vi "RemoteVI Next Free Port.vi"(0 "used":u16[](array[numeric]), 1 "start":u16=8100) -> (4 "port":u16)   [LabVIEW 2020, in "RemoteVI.lvlib"]
doc: "The first port from start up that none of used has (RemoteVI Server suggests it for the next share, used being the ports of RemoteVI Status.vi). Pure. Reference: nextFreePort() in tools\\lib\\server-app.mjs."
uses:
  RemoteVI.lvlib
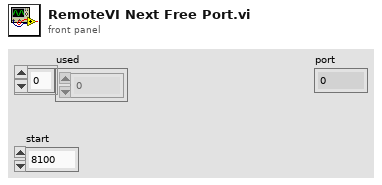
[diagram p1: front panel]
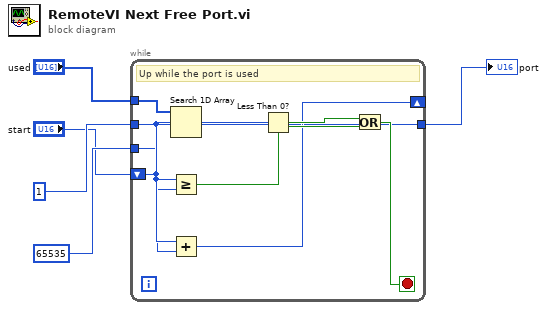
[diagram p0: block diagram]
diagram:
  n1 = while {
    tunnel: "used" -> [w6]
    tunnel: u16 1 -> [w7]
    tunnel: u16 65535 -> [w8]
    shift-right: [w10] -> _
    shift-left: "start" -> [w9]
    tunnel: [w9] -> w5
    stop <- w14 stop-if-true
    # "Up while the port is used"
    n2 = Search 1D Array(1D array=w6, element=w9) -> (index of element=w11:i32)  [unwired: 1 in]
    n3 = Greater Or Equal?(x=w9, y=w8) -> (x >= y?=w13:bool)
    n4 = Add(x=w9, y=w7) -> (x+y=w10:u16)
    n5 = Less Than 0?(x=w11) -> (x < 0?=w12:bool)
    n6 = Or(x=w12, y=w13) -> (x .or. y?=w14:bool)
  }
  "port" <- w5
